vi "EPC300x Utility Write To Register - Milliseconds.vi"(7 "Unit Address (1)":u8=1, 8 "error in (no error)":errorcluster, 9 "Data in ms (0)":u32, 10 "Register Address (0)":u16, 11 "VISA session":refnum<visa-resource-name>) -> (0 "error out":errorcluster, 3 "dup VISA session":refnum<visa-resource-name>)   [LabVIEW 2022 SP3]
doc: "This VI writes the values to the specified registers of specified unit."
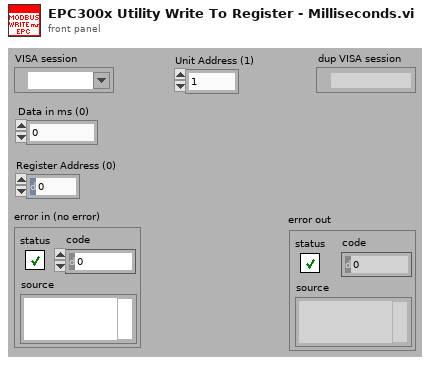
[diagram p1: front panel]
types:
  T1 = enum16{"By The Number of Bytes", "Copy Of the Sent Message"}
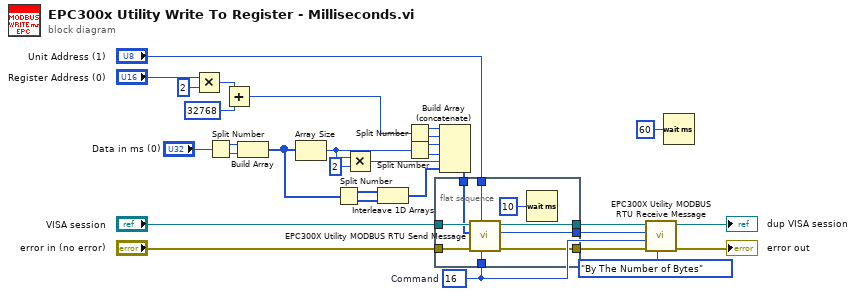
[diagram p0: block diagram]
diagram:
  w26 = u8 16  # Command
  n1 = Multiply(x="Register Address (0)", y=u16 2) -> (x*y=w8:u16)
  n2 = Split Number(x="Data in ms (0)") -> (hi(x)=w4:u16, lo(x)=w3:u16)
  n3 = Add(x=w8, y=u16 32768) -> (x+y=w5:u16)
  n4 = Build Array(w4, w3) -> (w10:u16[])
  n5 = Array Size(array=w10) -> (size(s)=w16:i32)
  n6 = Split Number(x=w10) -> (hi(x)=w12:u8[], lo(x)=w13:u8[])
  n7 = Multiply(x=w16, y=2) -> (x*y=w15:i32)
  n8 = Interleave 1D Arrays(w12, w13) -> (w11:u8[])
  n9 = Split Number(x=w5) -> (hi(x)=w24:u8, lo(x)=w23:u8)
  n10 = Split Number(x=w16) -> (hi(x)=w22:u16, lo(x)=w21:u16)
  n11 = flat-sequence {
    tunnel: "VISA session" -> [w40]
    tunnel: "error in (no error)" -> [w39]
    tunnel: [w38] -> w28
    tunnel: [w37] -> w27
    tunnel: w26 -> [w36]
    tunnel: w25 -> [w35]
    tunnel: [w34] -> w20
    tunnel: "Unit Address (1)" -> [w33]
    frame #0 {
      n12 = call "EPC300X Utility MODBUS RTU Send Message.vi"("Command (0)"=w36, "Unit Address (1)"=w33, "error in (no error)"=w39, "Message (empty array)"=w35, "VISA session"=w40) -> ("error out"=w38:errorcluster, "Length Of Sent MSG"=w34:u8, "dup VISA session"=w37:refnum<visa-resource-name>)  [unwired: 4 in]
      n13 = Wait (ms)(milliseconds to wait=u32 10) -> ()  [unwired: 1 out]
    }
  }
  n14 = Build Array (concatenate)(w24, w23, w22, w21, w15, w11) -> (w25:i32[])
  n15 = call "EPC300X Utility MODBUS RTU Receive Message.vi"("Receive Message Type (0: By The Number Of Bytes)"=T1."By The Number of Bytes" ("Receive Message Type"), "error in (no error)"=w28, "Sent Command (0)"=w26, "Length Of Sent MSG (0)"=w20, "VISA session"=w27) -> ("error out"=→"error out":errorcluster, "dup VISA session"=→"dup VISA session":refnum<visa-resource-name>)  [unwired: 4 in, 1 out]
  n16 = Wait (ms)(milliseconds to wait=u32 60) -> ()  [unwired: 1 out]
